vi "PC RC.vi"() -> ()   [LabVIEW 2017]
uses:
  <vilib>/Utility/inputDevices.llb/joystickAcquire.vi
  <vilib>/Utility/inputDevices.llb/closeJoystick.vi
panel:
  out "button 3":bool
  out "Z axis":i32
  in  "stop":bool
  out "pov 1":i32
  out "button 4":bool
  out "button 2":bool
  out "button 1":bool
  out "Y axis":i32
  out "X axis":i32
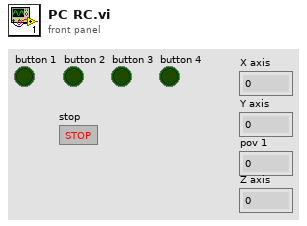
[diagram p1: front panel]
types:
  T1 = cluster{"X axis":i32, "Y axis":i32, "Z axis":i32, "X axis rotation":i32, "Y axis rotation":i32, "Z axis rotation":i32, "U axis":i32, "V axis":i32}
  T2 = cluster{"button 1":bool, "button 2":bool, "button 3":bool, "button 4":bool, "button 5":bool, "button 6":bool, "button 7":bool, "button 8":bool, "button 9":bool, "button 10":bool, "button 11":bool, "button 12":bool, "button 13":bool, "button 14":bool, "button 15":bool, "button 16":bool, "button 17":bool, "button 18":bool, "button 19":bool, "button 20":bool, "button 21":bool, "button 22":bool, "button 23":bool, "button 24":bool, "button 25":bool, "button 26":bool, "button 27":bool, "button 28":bool, "button 29":bool, "button 30":bool, "button 31":bool, "button 32":bool}
  T3 = cluster{"pov 1":i32, "pov 2":i32, "pov 3":i32, "pov 4":i32}
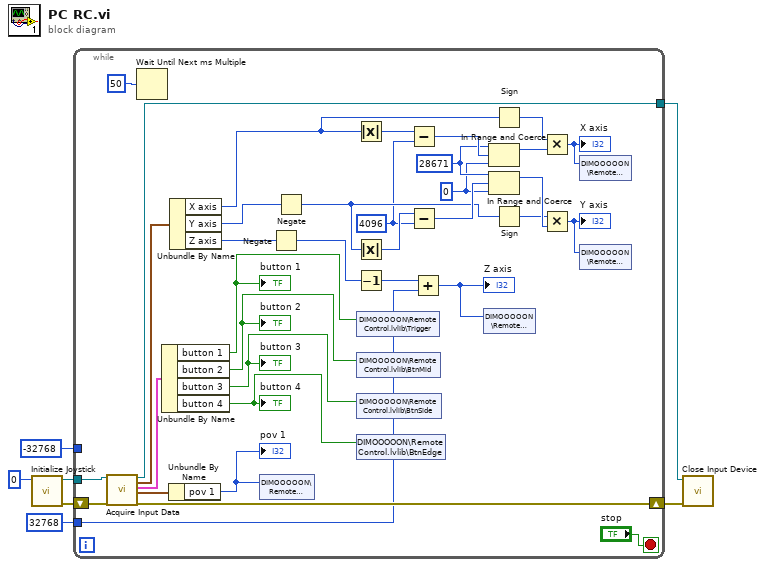
[diagram p0: block diagram]
diagram:
  n1 = call <vilib>:"Initialize Joystick.vi"("device index"=0) -> ("error out"=w5:errorcluster, "device ID"=w6:refnum<k1>)  [unwired: 9 in]
  n2 = while {
    tunnel: w6 -> [w42]
    shift-right: [w37] -> w4
    shift-left: w5 -> [w41]
    tunnel: [w36] -> w3
    tunnel: -32768 ("y") -> [_]
    tunnel: 32768 -> [w30]
    stop <- "stop" stop-if-true
    w12 = 0 ("upper limit")
    w13 = 28671 ("upper limit")
    w14 = 4096 ("y")
    n3 = call-poly <vilib>:"Acquire Input Data.vi"("device ID"=w42, "error in (no error)"=w41) -> ("device ID"=w36:refnum<k1>, "axis info"=w40:T1, "button info"=w39:T2, "direction info"=w38:T3, "error out"=w37:errorcluster)  [unwired: 13 in]
    n4 = Wait Until Next ms Multiple(millisecond multiple=u32 50) -> ()  [unwired: 1 out]
    n5 = Unbundle By Name(w39) -> ("button 1"=w32:bool, "button 2"=w33:bool, "button 3"=w8:bool, "button 4"=w9:bool)
    "button 1" <- w32
    "button 2" <- w33
    "button 4" <- w9
    "button 3" <- w8
    n6 = Unbundle By Name(w38) -> ("pov 1"=w34:i32)
    "pov 1" <- w34
    n7 = Unbundle By Name(w40) -> ("X axis"=w20:i32, "Y axis"=w25:i32, "Z axis"=w29:i32)
    n8 = shared-variable "DIMOOOOON\\Remote Control.lvlib\\LJ"(w34) -> ()  [unwired: 1 in, 1 out]
    n9 = Negate(x=w29) -> (-x=w27:i32)
    n10 = Negate(x=w25) -> (-x=w15:i32)
    n11 = Absolute Value(x=w20) -> (abs(x)=w24:i32)
    n12 = Absolute Value(x=w15) -> (abs(x)=w19:i32)
    n13 = Decrement(x=w27) -> (x-1=w26:i32)
    n14 = shared-variable "DIMOOOOON\\Remote Control.lvlib\\Trigger"(w32) -> ()  [unwired: 1 in, 1 out]
    n15 = shared-variable "DIMOOOOON\\Remote Control.lvlib\\BtnMid"(w33) -> ()  [unwired: 1 in, 1 out]
    n16 = shared-variable "DIMOOOOON\\Remote Control.lvlib\\BtnSide"(w8) -> ()  [unwired: 1 in, 1 out]
    n17 = shared-variable "DIMOOOOON\\Remote Control.lvlib\\BtnEdge"(w9) -> ()  [unwired: 1 in, 1 out]
    n18 = Subtract(x=w24, y=w14) -> (x-y=w23:i32)
    n19 = Subtract(x=w19, y=w14) -> (x-y=w18:i32)
    n20 = Add(x=w26, y=w30) -> (x+y=w28:i32)
    "Z axis" <- w28
    n21 = shared-variable "DIMOOOOON\\Remote Control.lvlib\\Z"(w28) -> ()  [unwired: 1 in, 1 out]
    n22 = In Range and Coerce(upper limit=w13, x=w23, lower limit=w12) -> (coerced(x)=w22:i32)  [unwired: 1 out]
    n23 = In Range and Coerce(upper limit=w13, x=w18, lower limit=w12) -> (coerced(x)=w17:i32)  [unwired: 1 out]
    n24 = Sign(1:w20) -> (0:w21:i32)
    n25 = Sign(1:w15) -> (0:w16:i32)
    n26 = Multiply(x=w21, y=w22) -> (x*y=w10:i32)
    "X axis" <- w10
    n27 = Multiply(x=w16, y=w17) -> (x*y=w11:i32)
    "Y axis" <- w11
    n28 = shared-variable "DIMOOOOON\\Remote Control.lvlib\\X"(w10) -> ()  [unwired: 1 in, 1 out]
    n29 = shared-variable "DIMOOOOON\\Remote Control.lvlib\\Y"(w11) -> ()  [unwired: 1 in, 1 out]
  }
  n30 = call-poly <vilib>:"Close Input Device.vi"("error in (no error)"=w4, "device ID"=w3) -> ()  [unwired: 8 in, 1 out]
